vi "auto_script_parser.vi"(7 "Tool Assignments":T1, 10 "Script name in":string="Script_1.txt", 11 "Script folder path":path=path "R:/Programing/Scriping/home/lvuser/auto") -> ()   [LabVIEW 2017, in "labview-standard-library.lvlib" / "automode-scripting.lvlib"]
uses:
  automode-scripting.lvlib
  footer/Footer_cluster.ctl
  type-defs/tool-assignments.ctl
  type-defs/command-statu-AE-control.ctl
panel:
  in  "Drive subsystem name":string="Drive"
  out "error out":errorcluster
  in  "Footer VI Cluster":T2
  out "File text out":string
  out "text":string
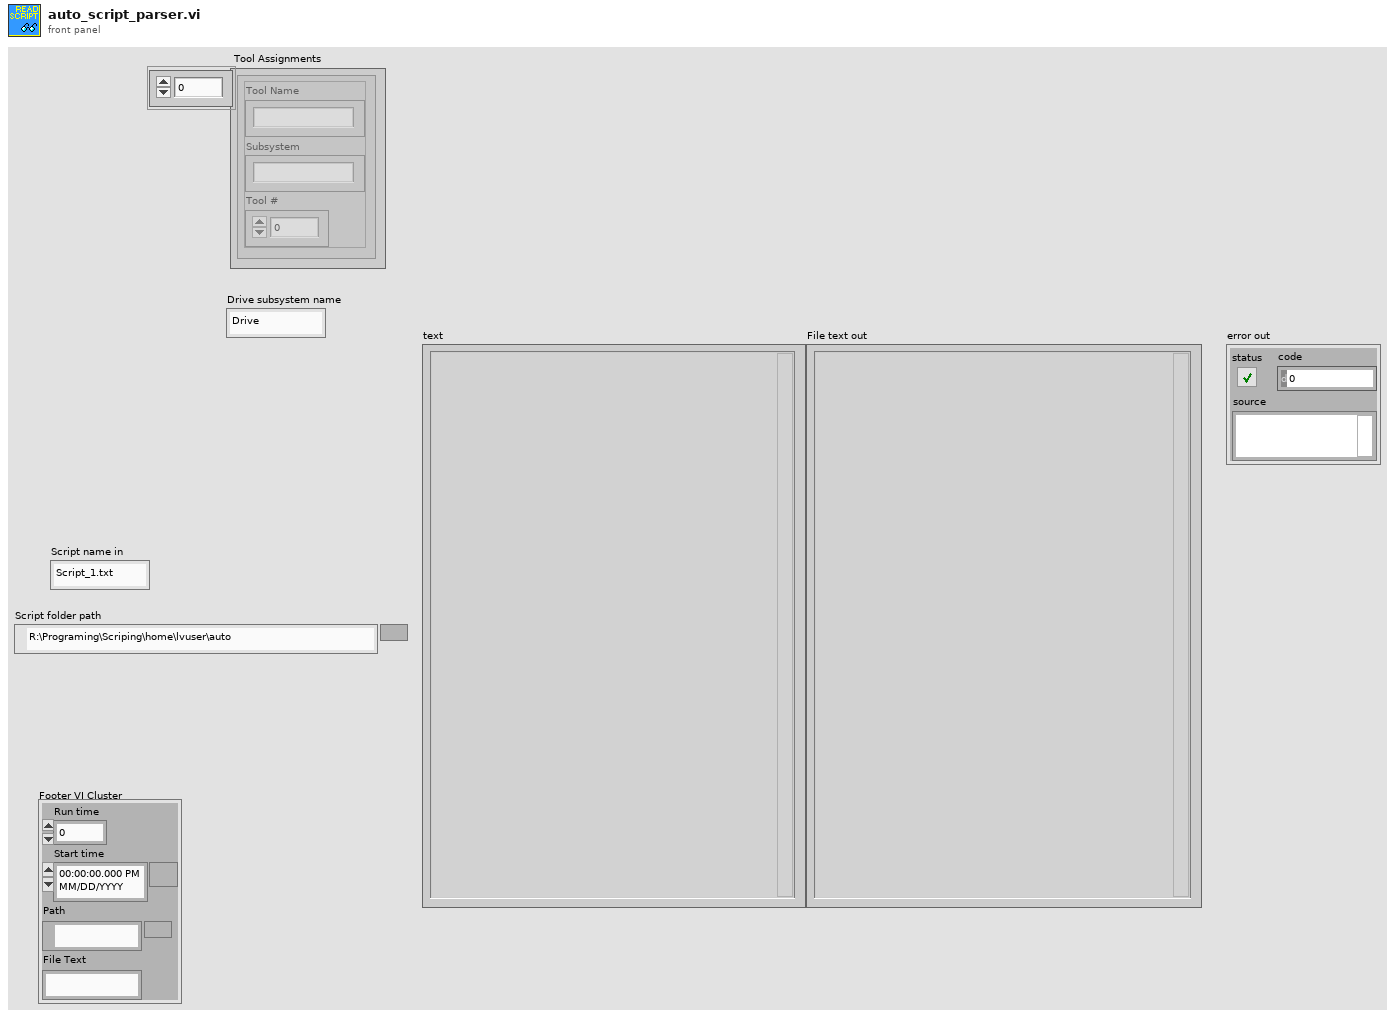
[diagram p1: front panel]
types:
  T1 = typedef "tool-assignments.ctl" = cluster{"Tool Name":string, "Subsystem":string, "Tool #":i32}[]
  T2 = typedef "labview-standard-library.lvlib/automode-scripting.lvlib/Footer_cluster.ctl" = cluster{"Run time":dbl, "Start time":timestamp, "Path":path, "File Text":string}
  T3 = typedef "command-statu-AE-control.ctl" = enum16{"Add to sent", "Add to complete", "Check last tool", "Check specific tool"}
  T4 = typedef "labview-standard-library.lvlib/automode-scripting.lvlib/code_types.ctl" = enum16{"g0", "g1", "g2", "g3", "g4", "g7", "m0", "m2", "tool", "comment"}
  T5 = typedef "labview-standard-library.lvlib/automode-scripting.lvlib/execution_stop_type.ctl" = enum16{"G4 timed pause", "G4 previous line pause", "G4 tool pause", "Invalid"}
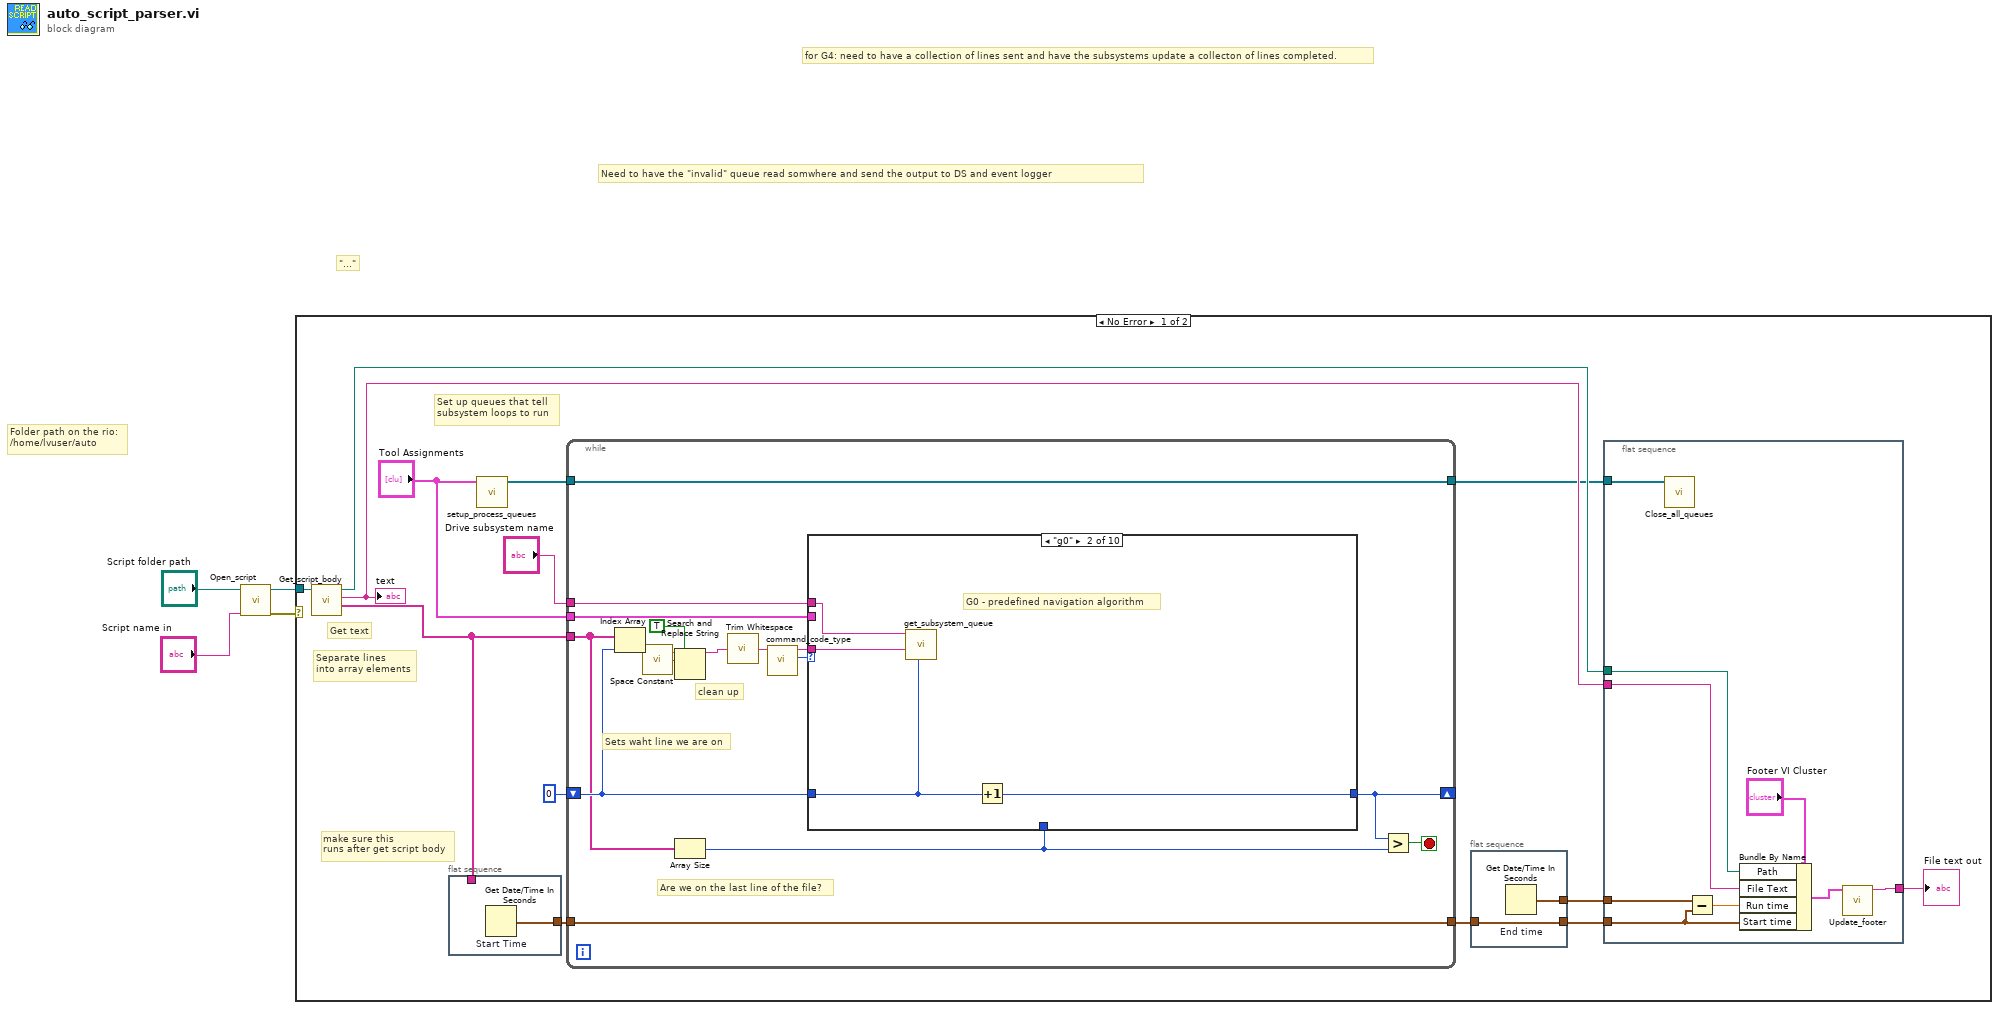
[diagram p0: block diagram]
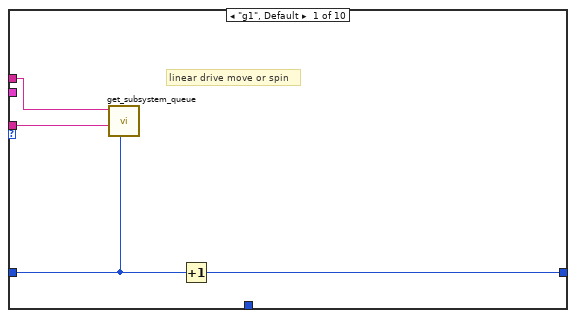
[diagram p2: hidden frame]
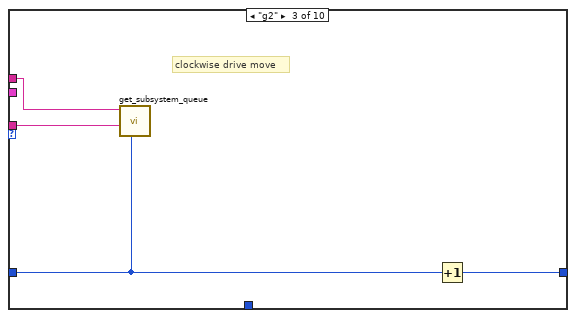
[diagram p3: hidden frame]
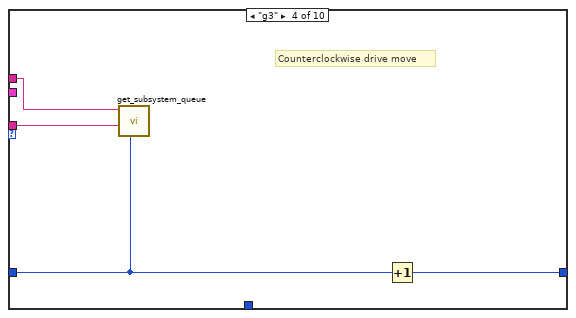
[diagram p4: hidden frame]
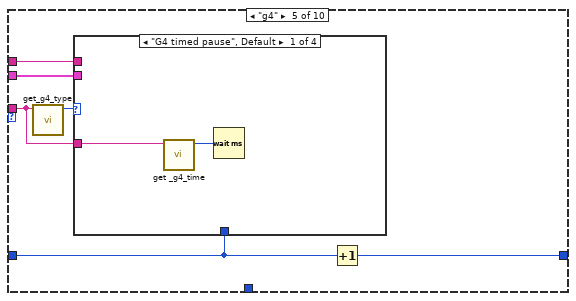
[diagram p5: hidden frame]
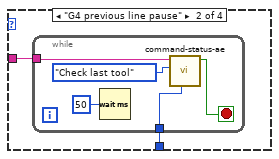
[diagram p6: hidden frame]
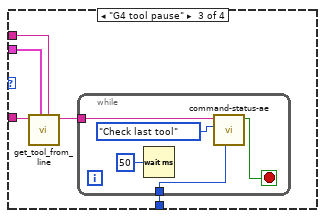
[diagram p7: hidden frame]
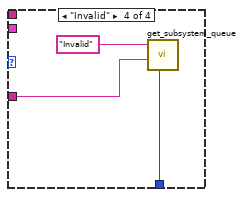
[diagram p8: hidden frame]
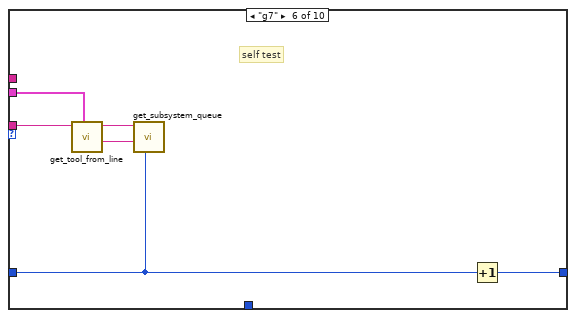
[diagram p9: hidden frame]
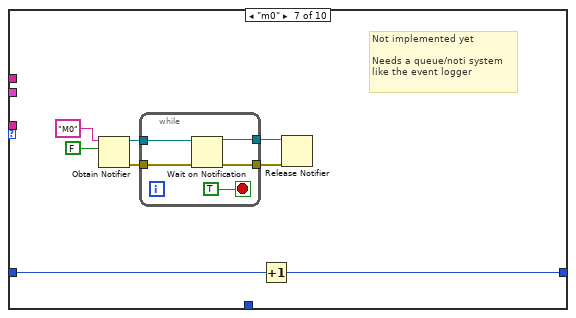
[diagram p10: hidden frame]
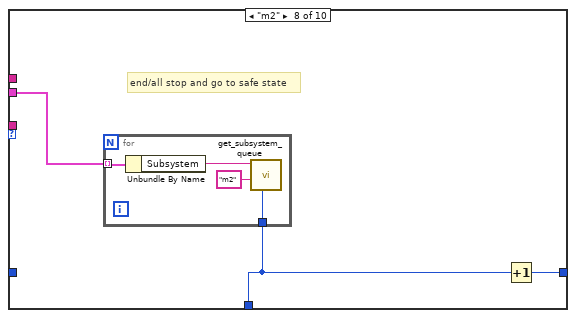
[diagram p11: hidden frame]
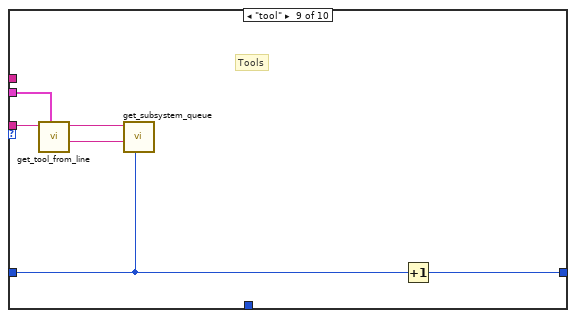
[diagram p12: hidden frame]
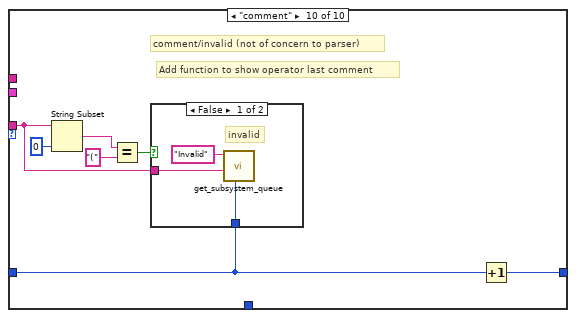
[diagram p13: hidden frame]
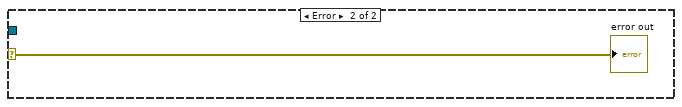
[diagram p15: hidden frame]
diagram:
  # "\"...\""
  # "for G4: need to have a collection of lines sent and have the subsystems update a collecton of lines completed."
  # "Need to have the \"invalid\" queue read somwhere and send the output to DS and event logger"
  # "Folder path on the rio:\n/home/lvuser/auto"
  n1 = call "Open_script.vi"("Script name"="Script name in", "Folder Path"="Script folder path") -> ("error out"=w2:errorcluster, "Byte Stream File out"=w1:refnum<file>)  [unwired: 8 in]
  n2 = case shown="No Error" w2 {
    selector: w2 -> [_ w133]
    tunnel: w1 -> [w17 _]
    frame No Error {
      # "make sure this\nruns after get script body"
      # "Get text"
      # "Set up queues that tell\nsubsystem loops to run"
      # "Separate lines\ninto array elements"
      n3 = call "Get_script_body.vi"("Byte Stream File in"=w17) -> ("Script Body"=w7:string[], "Full Text"=w14:string, "File Path Out"=w15:path)  [unwired: 8 in]
      "text" <- w14
      n4 = flat-sequence {
        tunnel: [w19] -> w16
        tunnel: w7 -> [_]
        frame #0 {
          n5 = Get Date/Time In Seconds "Start Time"() -> (seconds since 1Jan1904=w19:timestamp)
        }
      }
      n6 = call "setup_process_queues.vi"("Tool Assignments"="Tool Assignments") -> ("Process queues"=w12:refnum<queue>[])  [unwired: 9 in, 1 out]
      n7 = while {
        shift-right: [w45] -> _
        shift-left: 0 ("index") -> [w46]
        tunnel: w7 -> [w43]
        tunnel: w16 -> [w42]
        tunnel: [w42] -> w10
        tunnel: [w41] -> w11
        tunnel: w12 -> [w41]
        tunnel: "Tool Assignments" -> [w32]
        tunnel: "Drive subsystem name" -> [w31]
        stop <- w44 stop-if-true
        # "clean up"
        # "Are we on the last line of the file?"
        # "Sets waht line we are on"
        n8 = Index Array(array=w43, index=w46) -> (element=w36:string)
        n9 = call <vilib>:"Space Constant.vi"() -> ("String"=w38:string)
        n10 = Search and Replace String(replace all?=TRUE ("replace all? (F)"), input string=w36, search string=w38) -> (result string=w35:string)  [unwired: 5 in, 3 out]
        n11 = Array Size(array=w43) -> (size(s)=w33:i32)
        n12 = call <vilib>:"Trim Whitespace.vi"("string"=w35) -> ("trimmed string"=w34:string)  [unwired: 1 in]
        n13 = call "command_code_type.vi"("Line in"=w34) -> ("Code type out"=w40:T4, "Line out"=w39:string)  [unwired: 9 in]
        n14 = case shown="\"g0\"" w40 {
          tunnel: w46 -> [w48 w52 w56 w61 w65 w96 w104 _ w122 w123]
          tunnel: [w50 w54 w58 w60 w68 w95 w103 w112 w121 w129] -> w45
          tunnel: w39 -> [w49 w53 w57 w62 w66 w94 _ _ w120 w124]
          tunnel: w33 -> [_ _ _ _ _ _ _ w110 _ _]
          tunnel: w32 -> [_ _ _ _ w64 w93 _ w111 w119 _]
          tunnel: w31 -> [w47 w51 w55 w59 w63 _ _ _ _ _]
          frame "g1", Default {
            # "linear drive move or spin"
            n15 = call "get_subsystem_queue.vi"("Line #"=w48, "Line in"=w49, "Subsystem in"=w47) -> ()  [unwired: 9 in]
            n16 = Increment(x=w48) -> (x+1=w50:i32)
          }
          frame "g0" {
            # "G0 - predefined navigation algorithm"
            n17 = call "get_subsystem_queue.vi"("Line #"=w52, "Line in"=w53, "Subsystem in"=w51) -> ()  [unwired: 9 in]
            n18 = Increment(x=w52) -> (x+1=w54:i32)
          }
          frame "g2" {
            # "clockwise drive move"
            n19 = call "get_subsystem_queue.vi"("Line #"=w56, "Line in"=w57, "Subsystem in"=w55) -> ()  [unwired: 9 in]
            n20 = Increment(x=w56) -> (x+1=w58:i32)
          }
          frame "g3" {
            # "Counterclockwise drive move"
            n21 = call "get_subsystem_queue.vi"("Line #"=w61, "Line in"=w62, "Subsystem in"=w59) -> ()  [unwired: 9 in]
            n22 = Increment(x=w61) -> (x+1=w60:i32)
          }
          frame "g4" {
            n23 = call "get_g4_type.vi"("Line in"=w66) -> ("G4 type"=w67:T5)  [unwired: 9 in, 1 out]
            n24 = case shown="\"G4 timed pause\", Default" w67 {
              tunnel: w66 -> [w69 w72 w82 w90]
              tunnel: w65 -> [_ w71 w78 w89]
              tunnel: w64 -> [_ _ w81 _]
              tunnel: w63 -> [_ _ w80 _]
              frame "G4 timed pause", Default {
                n25 = call "get _g4_time.vi"("Line in"=w69) -> ("Time to wait"=w70:u32)  [unwired: 10 in]
                n26 = Wait (ms)(milliseconds to wait=w70) -> ()  [unwired: 1 out]
              }
              frame "G4 previous line pause" {
                n27 = while {
                  tunnel: w72 -> [w76]
                  tunnel: w71 -> [w73]
                  stop <- w75 stop-if-true
                  n28 = Wait (ms)(milliseconds to wait=u32 50) -> ()  [unwired: 1 out]
                  n29 = call "command-status-ae.vi"("line #"=w73, "ae command"=command-statu-AE-control."Check last tool", "tool# or drive subsystem name"=w76) -> ("Subsystem\ndone?"=w75:bool)  [unwired: 8 in]
                }
              }
              frame "G4 tool pause" {
                n30 = call "get_tool_from_line.vi"("Drive subsystem name"=w80, "Tool Assignments"=w81, "line in"=w82) -> ("Subsystem out"=w79:string)  [unwired: 7 in, 1 out]
                n31 = while {
                  tunnel: w79 -> [w86]
                  tunnel: w78 -> [w83]
                  stop <- w85 stop-if-true
                  n32 = Wait (ms)(milliseconds to wait=u32 50) -> ()  [unwired: 1 out]
                  n33 = call "command-status-ae.vi"("line #"=w83, "ae command"=command-statu-AE-control."Check last tool", "tool# or drive subsystem name"=w86) -> ("Subsystem\ndone?"=w85:bool)  [unwired: 8 in]
                }
              }
              frame "Invalid" {
                n34 = call "get_subsystem_queue.vi"("Line #"=w89, "Line in"=w90, "Subsystem in"="Invalid") -> ()  [unwired: 9 in]
              }
            }
            n35 = Increment(x=w65) -> (x+1=w68:i32)
          }
          frame "g7" {
            # "self test"
            n36 = call "get_tool_from_line.vi"("Tool Assignments"=w93, "line in"=w94) -> ("line out"=w91:string, "Subsystem out"=w92:string)  [unwired: 8 in]
            n37 = call "get_subsystem_queue.vi"("Line #"=w96, "Line in"=w91, "Subsystem in"=w92) -> ()  [unwired: 9 in]
            n38 = Increment(x=w96) -> (x+1=w95:i32)
          }
          frame "m0" {
            # "Not implemented yet\n\nNeeds a queue/noti system\nlike the event logger"
            n39 = Obtain Notifier(name (unnamed)="M0", notification data type=FALSE) -> (notifier out=w99:refnum<notifier>, error out=w100:errorcluster)  [unwired: 2 in, 1 out]
            n40 = while {
              tunnel: [w109] -> w102
              tunnel: [w108] -> w101
              tunnel: w100 -> [w107]
              tunnel: w99 -> [w106]
              stop <- TRUE stop-if-true
              n41 = Wait on Notification(notifier=w106, error in (no error)=w107) -> (notifier out=w109:refnum<notifier>, error out=w108:errorcluster)  [unwired: 2 in, 2 out]
            }
            n42 = Increment(x=w104) -> (x+1=w103:i32)
            n43 = Release Notifier(notifier=w102, error in (no error)=w101) -> ()  [unwired: 1 in, 3 out]
          }
          frame "m2" {
            # "end/all stop and go to safe state"
            n44 = for {
              tunnel: w111 -> [w115] mode=indexing
              tunnel: w110 -> [w116]
              n45 = Unbundle By Name(w115) -> ("Subsystem"=w114:string)
              n46 = call "get_subsystem_queue.vi"("Line #"=w116, "Line in"="m2", "Subsystem in"=w114) -> ()  [unwired: 9 in]
            }
            n47 = Increment(x=w110) -> (x+1=w112:i32)
          }
          frame "tool" {
            # "Tools"
            n48 = call "get_tool_from_line.vi"("Tool Assignments"=w119, "line in"=w120) -> ("line out"=w117:string, "Subsystem out"=w118:string)  [unwired: 8 in]
            n49 = call "get_subsystem_queue.vi"("Line #"=w122, "Line in"=w117, "Subsystem in"=w118) -> ()  [unwired: 9 in]
            n50 = Increment(x=w122) -> (x+1=w121:i32)
          }
          frame "comment" {
            # "Add function to show operator last comment"
            # "comment/invalid (not of concern to parser)"
            n51 = String Subset(string=w124, length (rest)=0 ("length (rest)")) -> (substring=w127:string)  [unwired: 1 in]
            n52 = Equal?(x=w127, y="(") -> (x = y?=w125:bool)
            n53 = case shown="False" w125 {
              tunnel: w124 -> [w131 _]
              tunnel: w123 -> [w130 _]
              frame False {
                # "invalid"
                n54 = call "get_subsystem_queue.vi"("Line #"=w130, "Line in"=w131, "Subsystem in"="Invalid") -> ()  [unwired: 9 in]
              }
              frame True {
                # "comment"
              }
            }
            n55 = Increment(x=w123) -> (x+1=w129:i32)
          }
        }
        n56 = Greater?(x=w45, y=w33) -> (0:w44:bool)
      }
      n57 = flat-sequence {
        tunnel: [w21] -> w9
        tunnel: w10 -> [w21]
        tunnel: [w20] -> w8
        frame #0 {
          n58 = Get Date/Time In Seconds "End time"() -> (seconds since 1Jan1904=w20:timestamp)
        }
      }
      n59 = flat-sequence {
        tunnel: w9 -> [w30]
        tunnel: w15 -> [w23]
        tunnel: w14 -> [w22]
        tunnel: [w29] -> w13
        tunnel: w11 -> [w24]
        tunnel: w8 -> [w25]
        frame #0 {
          n60 = call "Close_all_queues.vi"("Process queues"=w24) -> ()  [unwired: 11 in]
          n61 = Subtract(x=w25, y=w30) -> (x-y=w28:dbl)
          n62 = Bundle By Name(cluster="Footer VI Cluster", "Path"=w23, "File Text"=w22, "Run time"=w28, "Start time"=w30) -> (w26:T2)
          n63 = call "Update_footer.vi"("Footer info"=w26) -> ("File text out"=w29:string)  [unwired: 10 in]
        }
      }
      "File text out" <- w13
    }
    frame Error {
      "error out" <- w133
    }
  }
